vi "TT Move Test.vi"() -> ()   [LabVIEW 2023, in "Turn Table and Mast.lvlib" / "AUDIX EM1000.lvclass"]
uses:
  AUDIX EM1000.lvclass
  AUDIX EM1000.lvclass/AUDIX EM1000.ctl
panel:
  in  "Stop":bool
  out "TWL Limit Angle 2":string
  out "Current Angle after TWL 2":string
  out "number 2":i32
  out "number":i32
  in  "TT Speed":i32
  out "Current Angle after TWL":string
  out "TWL Limit Angle":string
  in  "VISA resource name":refnum<visa-resource-name>
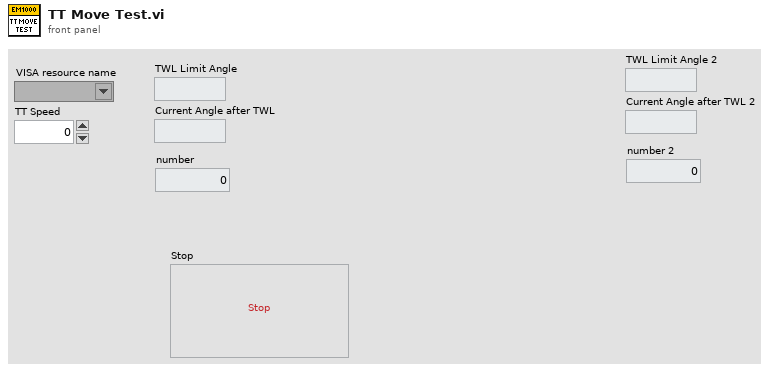
[diagram p1: front panel]
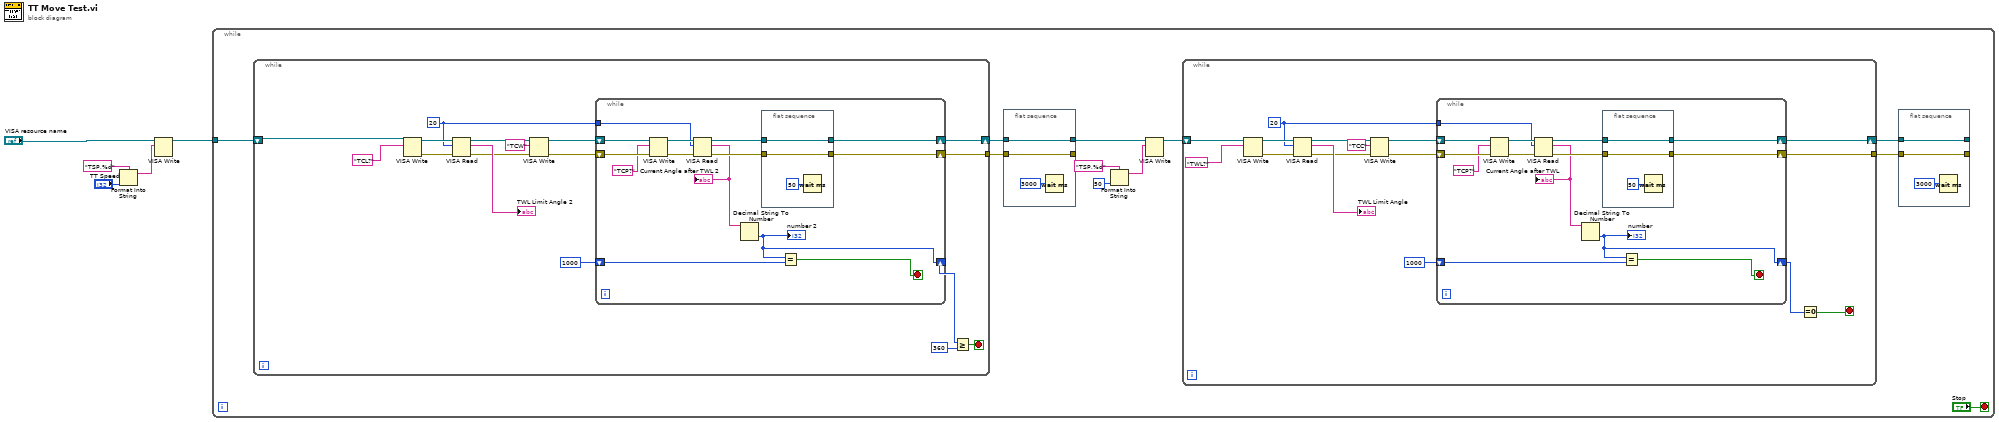
[diagram p0: block diagram]
diagram:
  n1 = Format Into String(format string="TSP,%d" ("포맷 문자열"), "TT Speed") -> (resulting string=w3:string)  [unwired: 2 in, 1 out]
  n2 = VISA Write(VISA resource name="VISA resource name", write buffer=w3) -> (VISA resource name out=w1:refnum<visa-resource-name>)  [unwired: 1 in, 2 out]
  n3 = while {
    tunnel: w1 -> [w14]
    stop <- "Stop" stop-if-true
    n4 = while {
      tunnel: [w28] -> w15
      shift-right: [w29] -> w16
      shift-left: w14 -> [w24]
      stop <- w25 stop-if-true
      w30 = u32 20 ("byte count")
      n5 = VISA Write(VISA resource name=w24, write buffer="TCL?") -> (VISA resource name out=w38:refnum<visa-resource-name>, error out=w37:errorcluster)  [unwired: 1 in, 1 out]
      n6 = VISA Read(VISA resource name=w38, byte count=w30, error in (no error)=w37) -> (VISA resource name out=w35:refnum<visa-resource-name>, read buffer=→"TWL Limit Angle 2":string, error out=w34:errorcluster)  [unwired: 1 out]
      n7 = VISA Write(VISA resource name=w35, write buffer="TCW", error in (no error)=w34) -> (VISA resource name out=w32:refnum<visa-resource-name>, error out=w31:errorcluster)  [unwired: 1 out]
      n8 = while {
        tunnel: w30 -> [w48]
        shift-right: [w45] -> w29
        shift-left: w32 -> [w53]
        shift-right: [w44] -> w28
        shift-left: w31 -> [w52]
        shift-right: [w41] -> w26
        shift-left: 1000 -> [w42]
        stop <- w40 stop-if-true
        n9 = VISA Write(VISA resource name=w53, write buffer="TCP?", error in (no error)=w52) -> (VISA resource name out=w50:refnum<visa-resource-name>, error out=w49:errorcluster)  [unwired: 1 out]
        n10 = VISA Read(VISA resource name=w50, byte count=w48, error in (no error)=w49) -> (VISA resource name out=w47:refnum<visa-resource-name>, read buffer=w43:string, error out=w46:errorcluster)  [unwired: 1 out]
        "Current Angle after TWL 2" <- w43
        n11 = Decimal String To Number(string=w43) -> (number=w41:i32)  [unwired: 2 in, 1 out]
        "number 2" <- w41
        n12 = flat-sequence {
          tunnel: w47 -> [w55]
          tunnel: w46 -> [w54]
          tunnel: [w55] -> w45
          tunnel: [w54] -> w44
          frame #0 {
            n13 = Wait (ms)(milliseconds to wait=u32 50) -> ()  [unwired: 1 out]
          }
        }
        n14 = Equal?(x=w41, y=w42) -> (x = y?=w40:bool)
      }
      n15 = Greater Or Equal?(x=w26, y=360) -> (x >= y?=w25:bool)
    }
    n16 = flat-sequence {
      tunnel: w16 -> [w21]
      tunnel: w15 -> [w20]
      tunnel: [w21] -> w8
      tunnel: [w20] -> _
      frame #0 {
        n17 = Wait (ms)(milliseconds to wait=u32 3000) -> ()  [unwired: 1 out]
      }
    }
    n18 = Format Into String(format string="TSP,%d" ("포맷 문자열"), 50 ("input 1")) -> (resulting string=w9:string)  [unwired: 2 in, 1 out]
    n19 = VISA Write(VISA resource name=w8, write buffer=w9) -> (VISA resource name out=w7:refnum<visa-resource-name>)  [unwired: 1 in, 2 out]
    n20 = while {
      tunnel: [w61] -> w12
      shift-right: [w62] -> w13
      shift-left: w7 -> [w60]
      stop <- w57 stop-if-true
      w63 = u32 20 ("byte count")
      n21 = VISA Write(VISA resource name=w60, write buffer="TWL?") -> (VISA resource name out=w71:refnum<visa-resource-name>, error out=w70:errorcluster)  [unwired: 1 in, 1 out]
      n22 = VISA Read(VISA resource name=w71, byte count=w63, error in (no error)=w70) -> (VISA resource name out=w68:refnum<visa-resource-name>, read buffer=→"TWL Limit Angle":string, error out=w67:errorcluster)  [unwired: 1 out]
      n23 = VISA Write(VISA resource name=w68, write buffer="TCC", error in (no error)=w67) -> (VISA resource name out=w65:refnum<visa-resource-name>, error out=w64:errorcluster)  [unwired: 1 out]
      n24 = while {
        tunnel: w63 -> [w81]
        shift-right: [w78] -> w62
        shift-left: w65 -> [w86]
        shift-right: [w77] -> w61
        shift-left: w64 -> [w85]
        shift-right: [w74] -> w58
        shift-left: 1000 -> [w75]
        stop <- w73 stop-if-true
        n25 = VISA Write(VISA resource name=w86, write buffer="TCP?", error in (no error)=w85) -> (VISA resource name out=w83:refnum<visa-resource-name>, error out=w82:errorcluster)  [unwired: 1 out]
        n26 = VISA Read(VISA resource name=w83, byte count=w81, error in (no error)=w82) -> (VISA resource name out=w80:refnum<visa-resource-name>, read buffer=w76:string, error out=w79:errorcluster)  [unwired: 1 out]
        "Current Angle after TWL" <- w76
        n27 = Decimal String To Number(string=w76) -> (number=w74:i32)  [unwired: 2 in, 1 out]
        "number" <- w74
        n28 = flat-sequence {
          tunnel: w80 -> [w88]
          tunnel: w79 -> [w87]
          tunnel: [w88] -> w78
          tunnel: [w87] -> w77
          frame #0 {
            n29 = Wait (ms)(milliseconds to wait=u32 50) -> ()  [unwired: 1 out]
          }
        }
        n30 = Equal?(x=w74, y=w75) -> (x = y?=w73:bool)
      }
      n31 = Equal To 0?(x=w58) -> (x = 0?=w57:bool)
    }
    n32 = flat-sequence {
      tunnel: w13 -> [w18]
      tunnel: w12 -> [w17]
      tunnel: [w18] -> _
      tunnel: [w17] -> _
      frame #0 {
        n33 = Wait (ms)(milliseconds to wait=u32 3000) -> ()  [unwired: 1 out]
      }
    }
  }
